vi "Backpressure test.vi"() -> ()   [LabVIEW 2021]
uses:
  typedef/Publisher Configuration.ctl
  typedef/Subscriber Configuration.ctl
  f27365a0-1864-4553-9f92-95bc83607519.vi
  57a9d767-a0aa-4728-95e7-aa61df6a1e2a.vi
  5d6ebc0a-921d-4227-9a00-435e824b8c93.vi
  d8bc2f99-22bc-43ae-b6fa-f8197ccb679b.vi
  1491cca6-a426-4f56-b87d-caac723d0473.vi
  39ed5927-df74-4a57-8dc9-96b021c80492.vi
  bbeb782f-bf74-416e-b0f9-de587b9af98f.vi
  859c98ed-807b-4b96-b06d-d6fb0e9e6f96.vi
  98931993-9e05-4946-a0e8-0782cf58acce.vi
  4db17f17-fbf3-42bc-8837-34dee5865092.vi
  ecbb9208-e776-414e-87f1-19c139091137.vi
  0167b3dc-6f49-4672-b3aa-d51916ebff2c.vi
  84c46a71-3ad6-417c-9aba-be379b5775e6.vi
  233ed9d6-ced9-42df-a9b8-edee980e2fa8.vi
  ff1f2ce0-8d1f-4625-a632-bddccbd44b74.vi
  06a3f26d-2d18-4b18-9314-4c38afe24da5.vi
  564cef77-d045-47f3-b68c-94ab523690b1.vi
  e3fe31ea-c0bd-4811-9f2d-7e19ce1afda0.vi
  23c5baeb-c843-4c9d-b5a5-34d50c9b2511.vi
  92b06e78-0e1e-4219-ba7d-c2e09868a523.vi
  SubVIs/Get Path.vi
  SubVIs/Convert Error.vi
  f27365a0-1864-4553-9f92-95bc83607519.vi/f164bb55-fadc-406a-97d8-e3295a396b46.vi
  SubVIs/Add Error.vi
  Refnum/Raw Publisher to Refnum.vi
  <vilib>/CIF Foundation/CIF Utilities/File/File/File Not Found Error Update.vi
  57a9d767-a0aa-4728-95e7-aa61df6a1e2a.vi/15451e88-64ef-462d-9cc0-58968935b893.vi
  Refnum/Raw Subscriber to Refnum.vi
  Refnum/Raw Publisher from Refnum.vi
  Refnum/Raw Subscriber from Refnum.vi
  1491cca6-a426-4f56-b87d-caac723d0473.vi/f164bb55-fadc-406a-97d8-e3295a396b46.vi
  39ed5927-df74-4a57-8dc9-96b021c80492.vi/15451e88-64ef-462d-9cc0-58968935b893.vi
  98931993-9e05-4946-a0e8-0782cf58acce.vi/f164bb55-fadc-406a-97d8-e3295a396b46.vi
  4db17f17-fbf3-42bc-8837-34dee5865092.vi/15451e88-64ef-462d-9cc0-58968935b893.vi
  84c46a71-3ad6-417c-9aba-be379b5775e6.vi/f164bb55-fadc-406a-97d8-e3295a396b46.vi
  ff1f2ce0-8d1f-4625-a632-bddccbd44b74.vi/15451e88-64ef-462d-9cc0-58968935b893.vi
  564cef77-d045-47f3-b68c-94ab523690b1.vi/f164bb55-fadc-406a-97d8-e3295a396b46.vi
  e3fe31ea-c0bd-4811-9f2d-7e19ce1afda0.vi/15451e88-64ef-462d-9cc0-58968935b893.vi
  <vilib>/Utility/error.llb/Trim Whitespace.vi
  SubVIs/Add Error Core.vi
  <vilib>/CIF Foundation/CIF Utilities/DataTypes/Utilities/Get Element Info of Variant.vi
  SubVIs/Get Type String.vi
  <vilib>/CIF Foundation/CIF Utilities/DataTypes/Utilities/Get JSON Descriptor of Variant.vi
  SubVIs/Convert Error Core.vi
  <vilib>/CIF Foundation/CIF Utilities/File/SubVIs/File Not Found Error Core.vi
  Iceoryx.lvlib
panel:
  out "status":string
  out "pass":bool
  out "error out":errorcluster
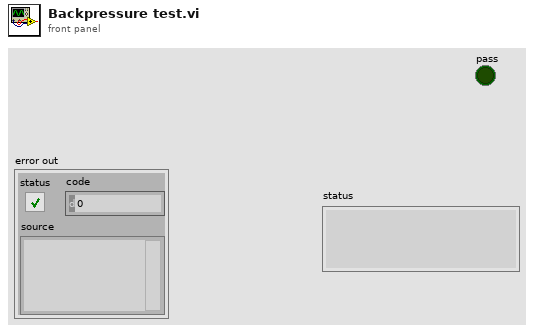
[diagram p1: front panel]
types:
  T1 = typedef "Iceoryx.lvlib/Subscriber Configuration.ctl" = cluster{"Name":string, "Topic":string, "Type":string, "Backpressure":bool}
  T2 = typedef "Iceoryx.lvlib/Publisher Configuration.ctl" = cluster{"Name":string, "Topic":string, "Type":string, "Best Effort Subscribers":u32, "Backpressure Subscribers":u32, "Best Effort Queue Depth":u32, "Backpressure Queue Depth":u32}
  T3 = typedef "Iceoryx.lvlib/Raw Publisher Refnum.ctl" = cluster{"refnum":u64, "Raw Pub":enum8{"rawpub"}}
  T4 = typedef "Iceoryx.lvlib/Raw Subscriber Refnum.ctl" = cluster{"refnum":u64, "Raw Sub":enum8{"rawsub"}}
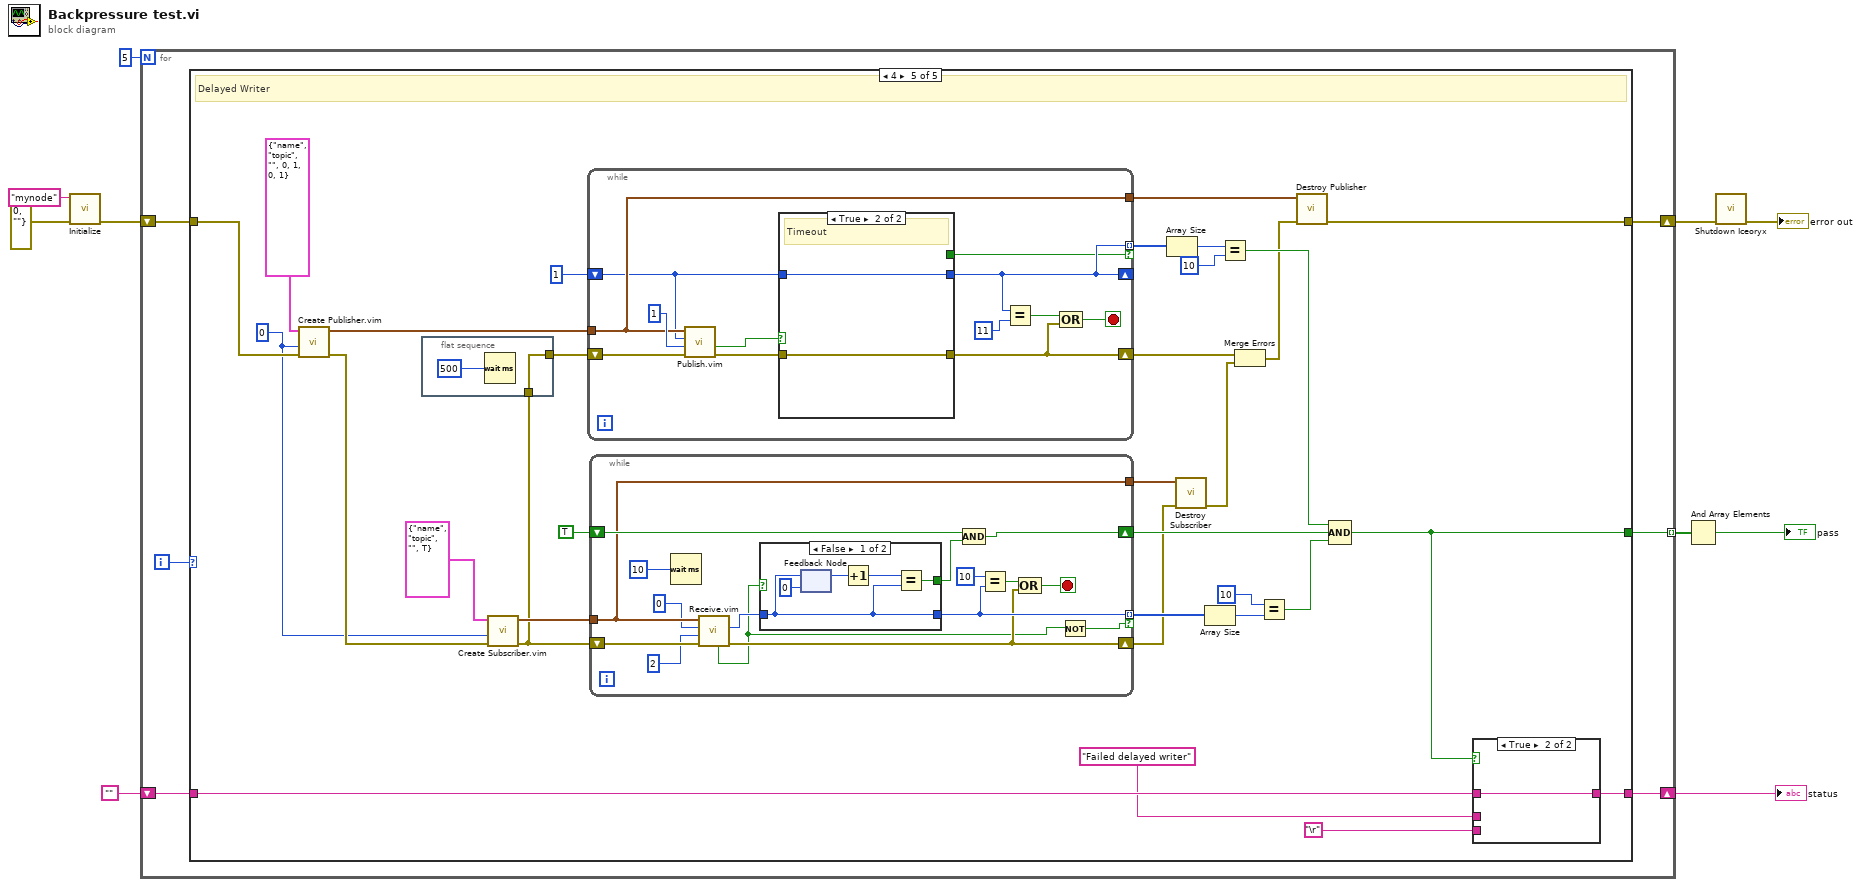
[diagram p0: block diagram]
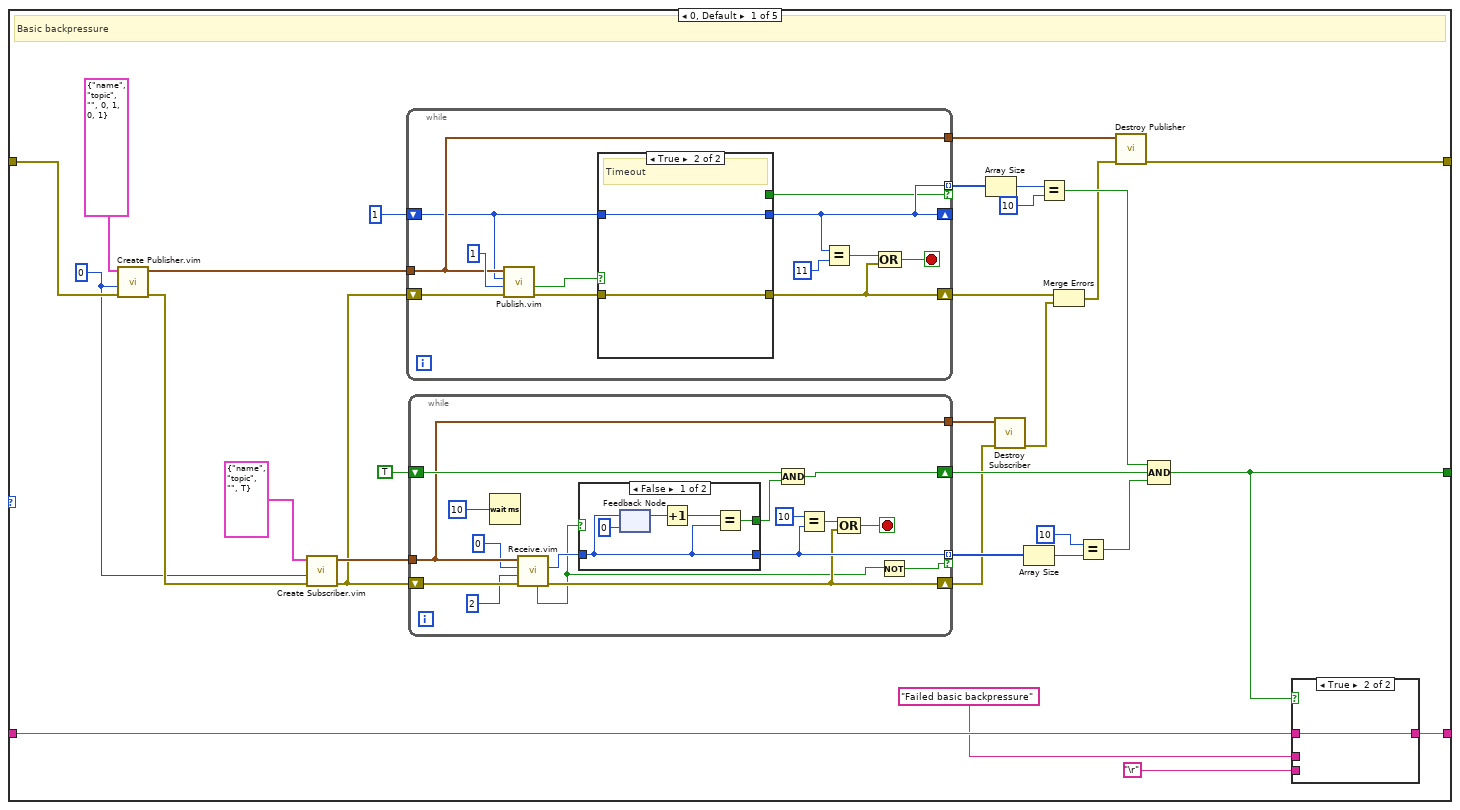
[diagram p2: hidden frame]
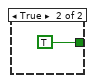
[diagram p3: hidden frame]
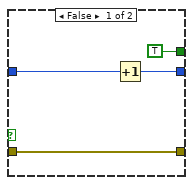
[diagram p4: hidden frame]
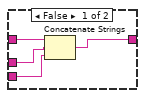
[diagram p5: hidden frame]
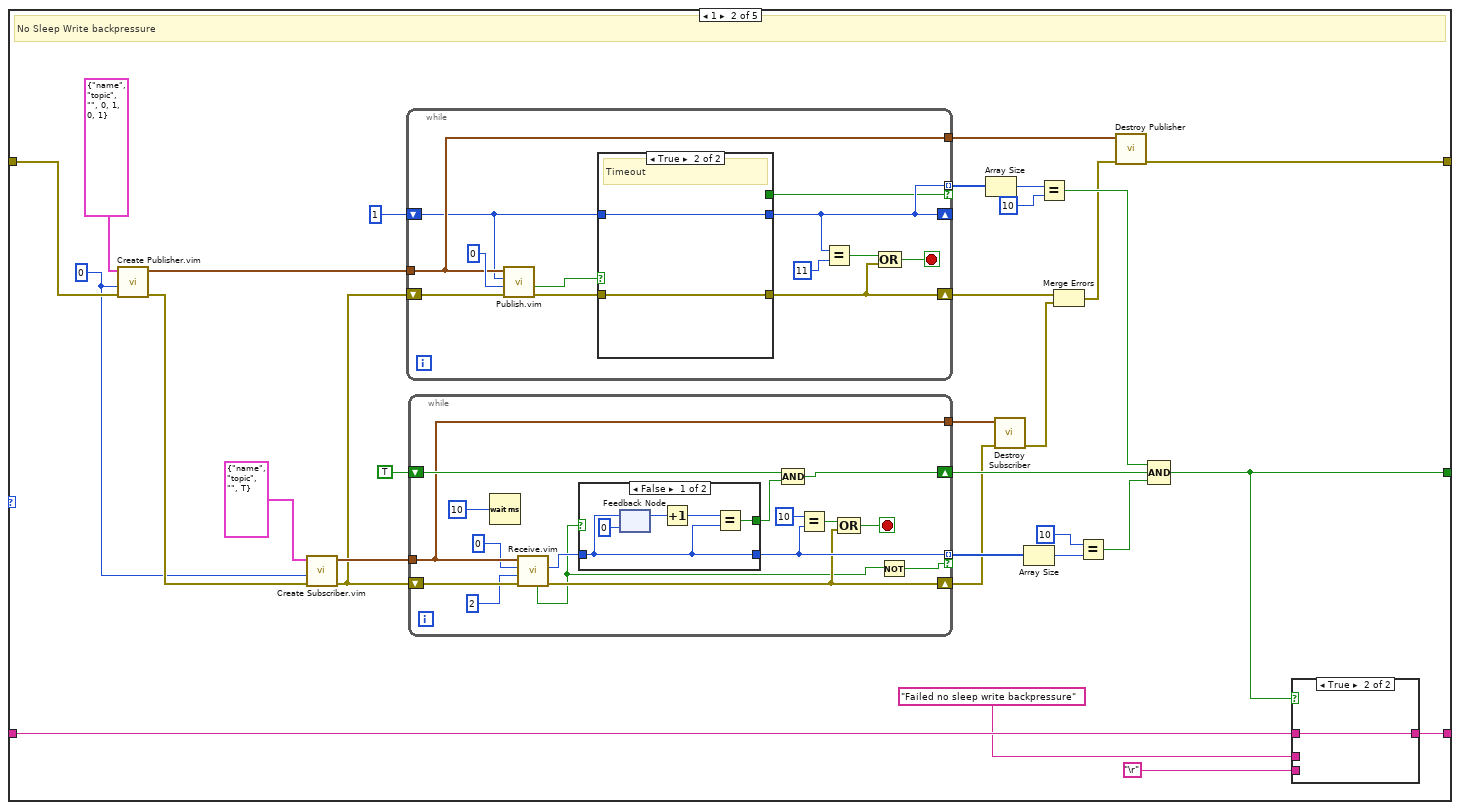
[diagram p6: hidden frame]
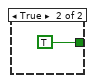
[diagram p7: hidden frame]
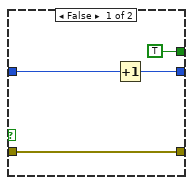
[diagram p8: hidden frame]
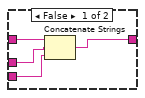
[diagram p9: hidden frame]
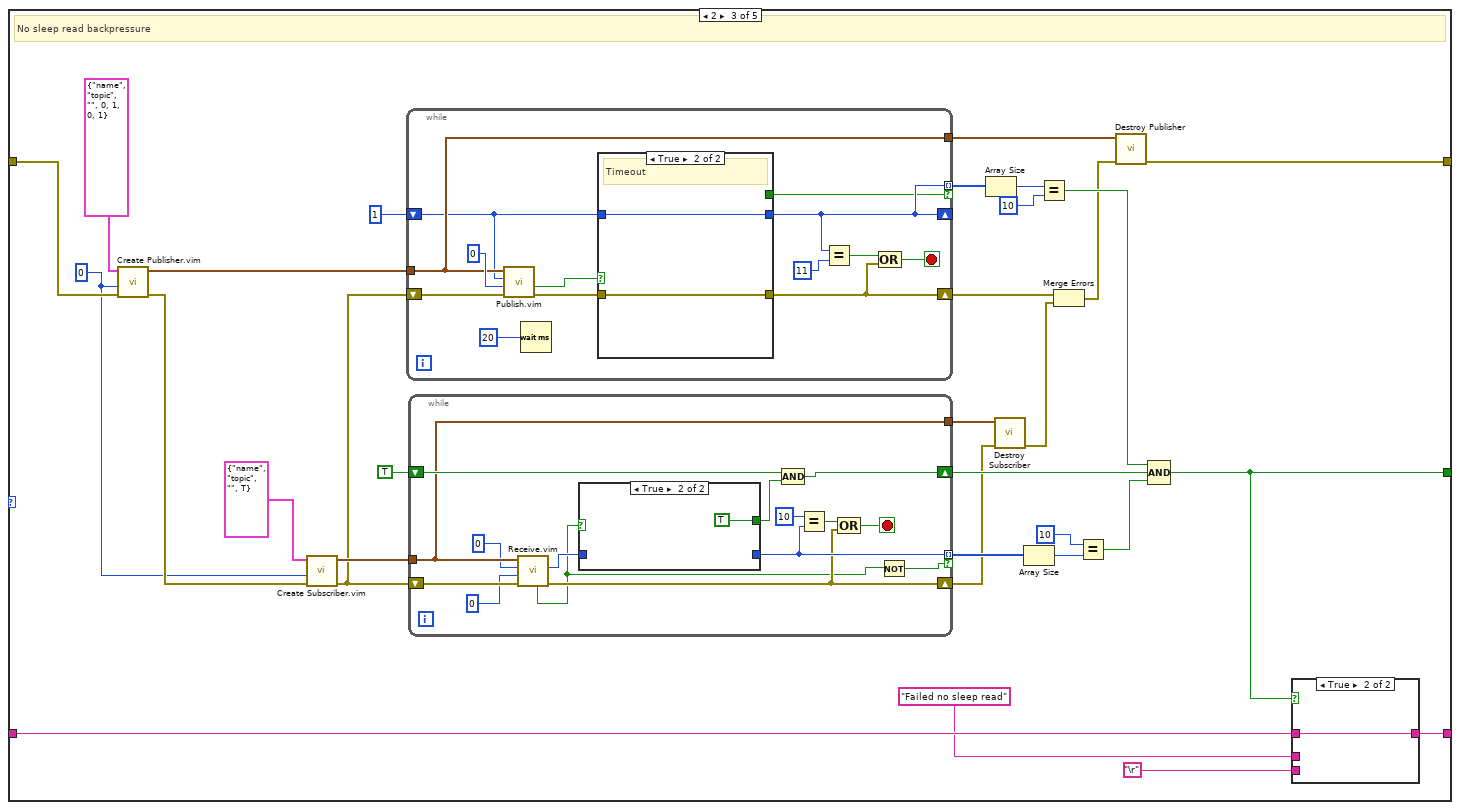
[diagram p10: hidden frame]
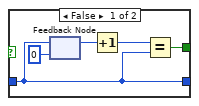
[diagram p11: hidden frame]
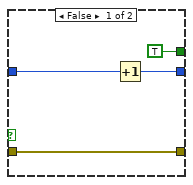
[diagram p12: hidden frame]
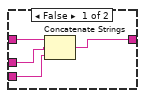
[diagram p13: hidden frame]
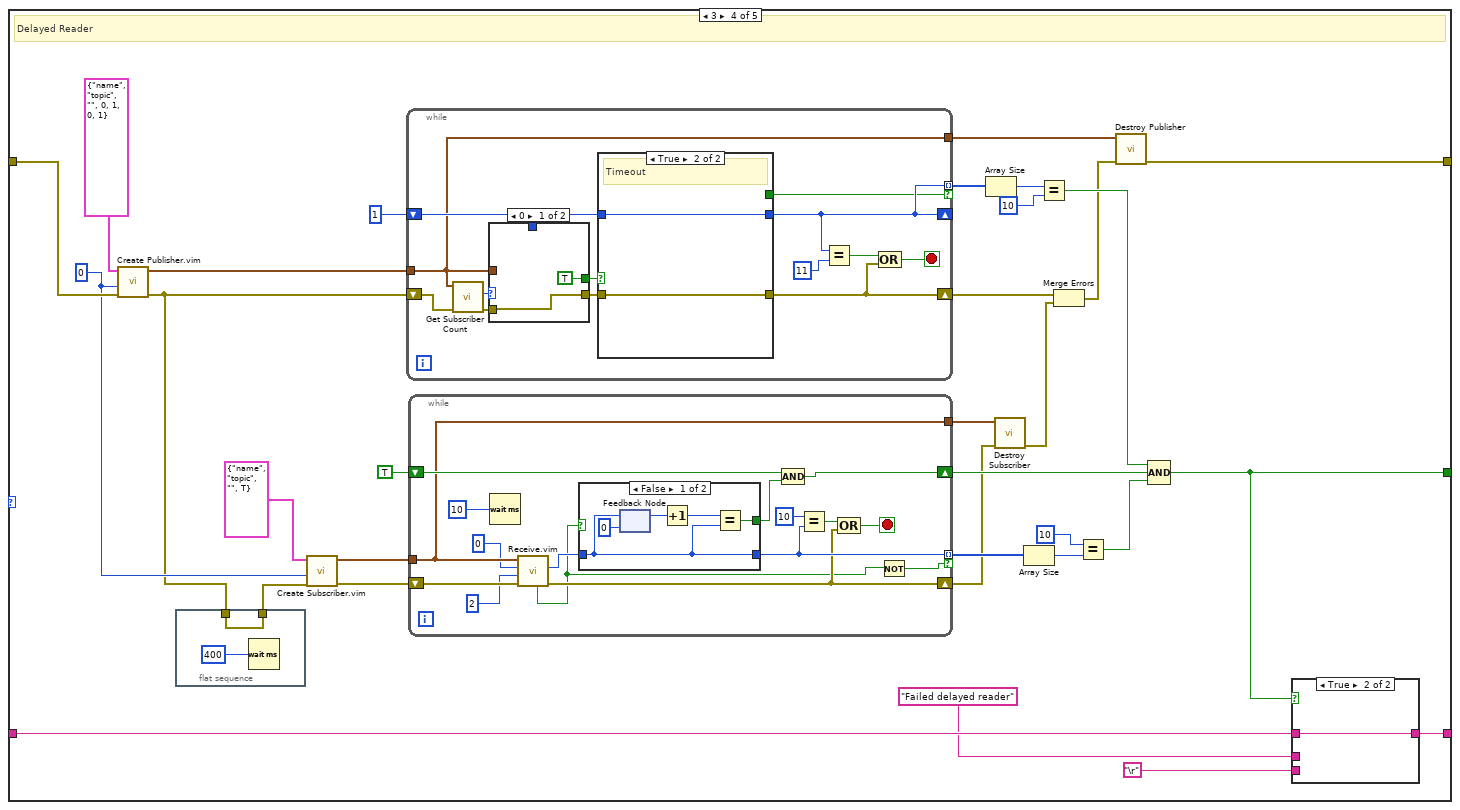
[diagram p14: hidden frame]
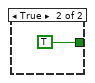
[diagram p15: hidden frame]
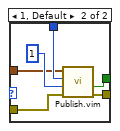
[diagram p16: hidden frame]
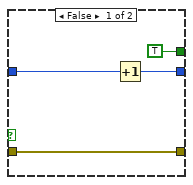
[diagram p17: hidden frame]
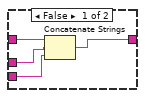
[diagram p18: hidden frame]
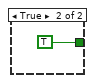
[diagram p19: hidden frame]
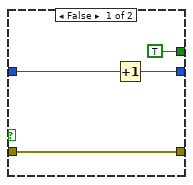
[diagram p20: hidden frame]
diagram:
  n1 = call "Initialize.vi"("error in (no error)"=errorcluster {"status"=FALSE, "code"=0, "source"=""} ("error out"), "Node name"="mynode") -> ("error out"=w4:errorcluster)  [unwired: 9 in]
  n2 = for {
    N: 5 -> [_]
    tunnel: [w16] -> w10 mode=indexing
    shift-right: [w13] -> w6
    shift-left: "" -> [w14]
    shift-right: [w12] -> w2
    shift-left: w4 -> [w11]
    i -> [w15]
    n3 = case shown="4" w15 {
      tunnel: [w35 w111 w187 w264 w352] -> w16
      tunnel: w14 -> [w47 w123 w199 w276 w364]
      tunnel: [w46 w122 w198 w275 w363] -> w13
      tunnel: [w18 w94 w170 w248 w335] -> w12
      tunnel: w11 -> [w30 w106 w182 w259 w347]
      frame 0, Default {
        w24 = 0
        # "Basic backpressure"
        n4 = call "Create Publisher.vim"("error in (no error)"=w30, "Data"=w24, "Publisher Configuration"=T2 {"Name"="name", "Topic"="topic", "Type"="", "Best Effort Subscribers"=0, "Backpressure Subscribers"=1, "Best Effort Queue Depth"=0, "Backpressure Queue Depth"=1}) -> ("error out"=w27:errorcluster, "Publisher Reference"=w28:T3)  [unwired: 6 in, 1 out]
        n5 = call "Create Subscriber.vim"("error in (no error)"=w27, "Data Type"=w24, "Subscriber Configuration"=T1 {"Name"="name", "Topic"="topic", "Type"="", "Backpressure"=TRUE}) -> ("error out"=w17:errorcluster, "Subscriber Reference"=w26:T4)  [unwired: 6 in, 1 out]
        n6 = while {
          tunnel: w28 -> [w72]
          shift-right: [w79] -> w43
          shift-left: w17 -> [w75]
          shift-right: [w77] -> _
          shift-left: 1 ("Data out") -> [w71]
          tunnel: [w77] -> w34 mode=indexing if=w76
          tunnel: [w72] -> w20
          stop <- w78 stop-if-true
          n7 = call "Publish.vim"("error in (no error)"=w75, "Timoeut ms"=i64 1 ("Timeout (ns)"), "Data In"=w71, "Publisher Reference"=w72) -> ("error out"=w70:errorcluster, "Timeout"=w73:bool)  [unwired: 5 in, 1 out]
          n8 = case shown="True" w73 {
            tunnel: w70 -> [w82 w87]
            tunnel: [w82 w87] -> w79
            tunnel: w71 -> [w85 w86]
            tunnel: [w84 w86] -> w77
            tunnel: [TRUE _] -> w76
            frame False {
              n9 = Increment(x=w85) -> (x+1=w84:i32)
            }
            frame True {
              # "Timeout"
            }
          }
          n10 = Equal?(x=w77, y=11) -> (x = y?=w80:bool)
          n11 = Compound Arithmetic op=OR(w80, w79) -> (w78:bool)
        }
        n12 = while {
          shift-right: [w60] -> w37
          shift-left: TRUE -> [w62]
          shift-right: [w53] -> w22
          shift-left: w17 -> [w55]
          tunnel: [w59] -> w40 mode=indexing if=w49
          tunnel: w26 -> [w54]
          tunnel: [w54] -> w23
          stop <- w56 stop-if-true
          n13 = Wait (ms)(milliseconds to wait=u32 10) -> ()  [unwired: 1 out]
          n14 = call "Receive.vim"("error in (no error)"=w55, "Timoeut ms"=2, "Data In"=0, "Subscriber Reference"=w54) -> ("error out"=w53:errorcluster, "Data Out"=w50:i32, "Timeout"=w48:bool)  [unwired: 4 in, 1 out]
          n15 = case shown="False" w48 {
            tunnel: w50 -> [w64 _]
            tunnel: [w65 TRUE] -> w61
            tunnel: [w64 _] -> w59
            frame False {
              n16 = feedback #1(0 ("Data out")) -> (w67:i32)
              n17 = feedback-in #1(w64) -> ()
              n18 = Increment(x=w67) -> (x+1=w66:i32)
              n19 = Equal?(x=w66, y=w64) -> (x = y?=w65:bool)
            }
            frame True {
            }
          }
          n20 = Compound Arithmetic op=AND(w62, w61) -> (w60:bool)
          n21 = Equal?(x=10, y=w59) -> (x = y?=w57:bool)
          n22 = Compound Arithmetic op=OR(w57, w53) -> (w56:bool)
          n23 = Not(x=w48) -> (.not. x?=w49:bool)
        }
        n24 = Array Size(array=w34) -> (size(s)=w33:i32)
        n25 = call "Destroy Subscriber.vi"("error in (no error)"=w22, "Subscriber Reference"=w23) -> ("error out"=w21:errorcluster)  [unwired: 9 in]
        n26 = Array Size(array=w40) -> (size(s)=w39:i32)
        n27 = Equal?(x=w33, y=10 ("x")) -> (x = y?=w31:bool)
        n28 = Merge Errors(w43, w21) -> (w19:errorcluster)
        n29 = Equal?(x=10, y=w39) -> (x = y?=w36:bool)
        n30 = call "Destroy Publisher.vi"("error in (no error)"=w19, "Publisher Reference"=w20) -> ("error out"=w18:errorcluster)  [unwired: 9 in]
        n31 = Compound Arithmetic op=AND(w31, w37, w36) -> (w35:bool)
        n32 = case shown="True" w35 {
          tunnel: w47 -> [w91 w92]
          tunnel: [w88 w92] -> w46
          tunnel: "Failed basic backpressure" -> [w90 _]
          tunnel: "\r" -> [w89 _]
          frame False {
            n33 = Concatenate Strings(w91, w90, w89) -> (w88:string)
          }
          frame True {
          }
        }
      }
      frame 1 {
        w100 = 0
        # "No Sleep Write backpressure"
        n34 = call "Create Publisher.vim"("error in (no error)"=w106, "Data"=w100, "Publisher Configuration"=T2 {"Name"="name", "Topic"="topic", "Type"="", "Best Effort Subscribers"=0, "Backpressure Subscribers"=1, "Best Effort Queue Depth"=0, "Backpressure Queue Depth"=1}) -> ("error out"=w103:errorcluster, "Publisher Reference"=w104:T3)  [unwired: 6 in, 1 out]
        n35 = call "Create Subscriber.vim"("error in (no error)"=w103, "Data Type"=w100, "Subscriber Configuration"=T1 {"Name"="name", "Topic"="topic", "Type"="", "Backpressure"=TRUE}) -> ("error out"=w93:errorcluster, "Subscriber Reference"=w102:T4)  [unwired: 6 in, 1 out]
        n36 = while {
          tunnel: w104 -> [w148]
          shift-right: [w155] -> w119
          shift-left: w93 -> [w151]
          shift-right: [w153] -> _
          shift-left: 1 ("Data out") -> [w147]
          tunnel: [w153] -> w110 mode=indexing if=w152
          tunnel: [w148] -> w96
          stop <- w154 stop-if-true
          n37 = call "Publish.vim"("error in (no error)"=w151, "Timoeut ms"=i64 0 ("Timeout (ns)"), "Data In"=w147, "Publisher Reference"=w148) -> ("error out"=w146:errorcluster, "Timeout"=w149:bool)  [unwired: 5 in, 1 out]
          n38 = case shown="True" w149 {
            tunnel: w146 -> [w158 w163]
            tunnel: [w158 w163] -> w155
            tunnel: w147 -> [w161 w162]
            tunnel: [w160 w162] -> w153
            tunnel: [TRUE _] -> w152
            frame False {
              n39 = Increment(x=w161) -> (x+1=w160:i32)
            }
            frame True {
              # "Timeout"
            }
          }
          n40 = Equal?(x=w153, y=11) -> (x = y?=w156:bool)
          n41 = Compound Arithmetic op=OR(w156, w155) -> (w154:bool)
        }
        n42 = while {
          shift-right: [w136] -> w113
          shift-left: TRUE -> [w138]
          shift-right: [w129] -> w98
          shift-left: w93 -> [w131]
          tunnel: [w135] -> w116 mode=indexing if=w125
          tunnel: w102 -> [w130]
          tunnel: [w130] -> w99
          stop <- w132 stop-if-true
          n43 = Wait (ms)(milliseconds to wait=u32 10) -> ()  [unwired: 1 out]
          n44 = call "Receive.vim"("error in (no error)"=w131, "Timoeut ms"=2, "Data In"=0, "Subscriber Reference"=w130) -> ("error out"=w129:errorcluster, "Data Out"=w126:i32, "Timeout"=w124:bool)  [unwired: 4 in, 1 out]
          n45 = case shown="False" w124 {
            tunnel: w126 -> [w140 _]
            tunnel: [w141 TRUE] -> w137
            tunnel: [w140 _] -> w135
            frame False {
              n46 = feedback #2(0 ("Data out")) -> (w143:i32)
              n47 = feedback-in #2(w140) -> ()
              n48 = Increment(x=w143) -> (x+1=w142:i32)
              n49 = Equal?(x=w142, y=w140) -> (x = y?=w141:bool)
            }
            frame True {
            }
          }
          n50 = Compound Arithmetic op=AND(w138, w137) -> (w136:bool)
          n51 = Equal?(x=10, y=w135) -> (x = y?=w133:bool)
          n52 = Compound Arithmetic op=OR(w133, w129) -> (w132:bool)
          n53 = Not(x=w124) -> (.not. x?=w125:bool)
        }
        n54 = Array Size(array=w110) -> (size(s)=w109:i32)
        n55 = call "Destroy Subscriber.vi"("error in (no error)"=w98, "Subscriber Reference"=w99) -> ("error out"=w97:errorcluster)  [unwired: 9 in]
        n56 = Array Size(array=w116) -> (size(s)=w115:i32)
        n57 = Equal?(x=w109, y=10 ("x")) -> (x = y?=w107:bool)
        n58 = Merge Errors(w119, w97) -> (w95:errorcluster)
        n59 = Equal?(x=10, y=w115) -> (x = y?=w112:bool)
        n60 = call "Destroy Publisher.vi"("error in (no error)"=w95, "Publisher Reference"=w96) -> ("error out"=w94:errorcluster)  [unwired: 9 in]
        n61 = Compound Arithmetic op=AND(w107, w113, w112) -> (w111:bool)
        n62 = case shown="True" w111 {
          tunnel: w123 -> [w167 w168]
          tunnel: [w164 w168] -> w122
          tunnel: "Failed no sleep write backpressure" -> [w166 _]
          tunnel: "\r" -> [w165 _]
          frame False {
            n63 = Concatenate Strings(w167, w166, w165) -> (w164:string)
          }
          frame True {
          }
        }
      }
      frame 2 {
        w176 = 0
        # "No sleep read backpressure"
        n64 = call "Create Publisher.vim"("error in (no error)"=w182, "Data"=w176, "Publisher Configuration"=T2 {"Name"="name", "Topic"="topic", "Type"="", "Best Effort Subscribers"=0, "Backpressure Subscribers"=1, "Best Effort Queue Depth"=0, "Backpressure Queue Depth"=1}) -> ("error out"=w179:errorcluster, "Publisher Reference"=w180:T3)  [unwired: 6 in, 1 out]
        n65 = call "Create Subscriber.vim"("error in (no error)"=w179, "Data Type"=w176, "Subscriber Configuration"=T1 {"Name"="name", "Topic"="topic", "Type"="", "Backpressure"=TRUE}) -> ("error out"=w169:errorcluster, "Subscriber Reference"=w178:T4)  [unwired: 6 in, 1 out]
        n66 = while {
          tunnel: w180 -> [w224]
          shift-right: [w231] -> w195
          shift-left: w169 -> [w227]
          shift-right: [w229] -> _
          shift-left: 1 ("Data out") -> [w223]
          tunnel: [w229] -> w186 mode=indexing if=w228
          tunnel: [w224] -> w172
          stop <- w230 stop-if-true
          n67 = call "Publish.vim"("error in (no error)"=w227, "Timoeut ms"=i64 0 ("Timeout (ns)"), "Data In"=w223, "Publisher Reference"=w224) -> ("error out"=w222:errorcluster, "Timeout"=w225:bool)  [unwired: 5 in, 1 out]
          n68 = Wait (ms)(milliseconds to wait=u32 20) -> ()  [unwired: 1 out]
          n69 = case shown="True" w225 {
            tunnel: w222 -> [w234 w239]
            tunnel: [w234 w239] -> w231
            tunnel: w223 -> [w237 w238]
            tunnel: [w236 w238] -> w229
            tunnel: [TRUE _] -> w228
            frame False {
              n70 = Increment(x=w237) -> (x+1=w236:i32)
            }
            frame True {
              # "Timeout"
            }
          }
          n71 = Equal?(x=w229, y=11) -> (x = y?=w232:bool)
          n72 = Compound Arithmetic op=OR(w232, w231) -> (w230:bool)
        }
        n73 = while {
          shift-right: [w212] -> w189
          shift-left: TRUE -> [w214]
          shift-right: [w205] -> w174
          shift-left: w169 -> [w207]
          tunnel: [w211] -> w192 mode=indexing if=w201
          tunnel: w178 -> [w206]
          tunnel: [w206] -> w175
          stop <- w208 stop-if-true
          n74 = call "Receive.vim"("error in (no error)"=w207, "Timoeut ms"=0, "Data In"=0, "Subscriber Reference"=w206) -> ("error out"=w205:errorcluster, "Data Out"=w202:i32, "Timeout"=w200:bool)  [unwired: 4 in, 1 out]
          n75 = case shown="True" w200 {
            tunnel: w202 -> [w215 _]
            tunnel: [w216 TRUE] -> w213
            tunnel: [w215 _] -> w211
            frame False {
              n76 = feedback #3(0 ("Data out")) -> (w218:i32)
              n77 = feedback-in #3(w215) -> ()
              n78 = Increment(x=w218) -> (x+1=w217:i32)
              n79 = Equal?(x=w217, y=w215) -> (x = y?=w216:bool)
            }
            frame True {
            }
          }
          n80 = Compound Arithmetic op=AND(w214, w213) -> (w212:bool)
          n81 = Equal?(x=10, y=w211) -> (x = y?=w209:bool)
          n82 = Compound Arithmetic op=OR(w209, w205) -> (w208:bool)
          n83 = Not(x=w200) -> (.not. x?=w201:bool)
        }
        n84 = Array Size(array=w186) -> (size(s)=w185:i32)
        n85 = call "Destroy Subscriber.vi"("error in (no error)"=w174, "Subscriber Reference"=w175) -> ("error out"=w173:errorcluster)  [unwired: 9 in]
        n86 = Array Size(array=w192) -> (size(s)=w191:i32)
        n87 = Equal?(x=w185, y=10 ("x")) -> (x = y?=w183:bool)
        n88 = Merge Errors(w195, w173) -> (w171:errorcluster)
        n89 = Equal?(x=10, y=w191) -> (x = y?=w188:bool)
        n90 = call "Destroy Publisher.vi"("error in (no error)"=w171, "Publisher Reference"=w172) -> ("error out"=w170:errorcluster)  [unwired: 9 in]
        n91 = Compound Arithmetic op=AND(w183, w189, w188) -> (w187:bool)
        n92 = case shown="True" w187 {
          tunnel: w199 -> [w243 w244]
          tunnel: [w240 w244] -> w198
          tunnel: "Failed no sleep read" -> [w242 _]
          tunnel: "\r" -> [w241 _]
          frame False {
            n93 = Concatenate Strings(w243, w242, w241) -> (w240:string)
          }
          frame True {
          }
        }
      }
      frame 3 {
        w254 = 0
        # "Delayed Reader"
        n94 = call "Create Publisher.vim"("error in (no error)"=w259, "Data"=w254, "Publisher Configuration"=T2 {"Name"="name", "Topic"="topic", "Type"="", "Best Effort Subscribers"=0, "Backpressure Subscribers"=1, "Best Effort Queue Depth"=0, "Backpressure Queue Depth"=1}) -> ("error out"=w245:errorcluster, "Publisher Reference"=w257:T3)  [unwired: 6 in, 1 out]
        n95 = flat-sequence {
          tunnel: w245 -> [w278]
          tunnel: [w278] -> w246
          frame #0 {
            n96 = Wait (ms)(milliseconds to wait=u32 400) -> ()  [unwired: 1 out]
          }
        }
        n97 = call "Create Subscriber.vim"("error in (no error)"=w246, "Data Type"=w254, "Subscriber Configuration"=T1 {"Name"="name", "Topic"="topic", "Type"="", "Backpressure"=TRUE}) -> ("error out"=w247:errorcluster, "Subscriber Reference"=w256:T4)  [unwired: 6 in, 1 out]
        n98 = while {
          tunnel: w257 -> [w304]
          shift-right: [w311] -> w272
          shift-left: w245 -> [w303]
          shift-right: [w309] -> _
          shift-left: 1 ("Data out") -> [w306]
          tunnel: [w309] -> w263 mode=indexing if=w308
          tunnel: [w304] -> w250
          stop <- w310 stop-if-true
          n99 = call "Get Subscriber Count.vi"("error in (no error)"=w303, "Publisher Reference"=w304) -> ("error out"=w302:errorcluster, "Backpressure"=w301:u32)  [unwired: 7 in, 1 out]
          n100 = case shown="0" w301 {
            tunnel: [TRUE ("Timeout") w320] -> w307
            tunnel: w306 -> [_ w319]
            tunnel: [w315 w318] -> w305
            tunnel: w304 -> [_ w317]
            tunnel: w302 -> [w315 w316]
            frame 0 {
            }
            frame 1, Default {
              n101 = call "Publish.vim"("error in (no error)"=w316, "Timoeut ms"=i64 1 ("Timeout (ns)"), "Data In"=w319, "Publisher Reference"=w317) -> ("error out"=w318:errorcluster, "Timeout"=w320:bool)  [unwired: 5 in, 1 out]
            }
          }
          n102 = case shown="True" w307 {
            tunnel: w305 -> [w322 w327]
            tunnel: [w322 w327] -> w311
            tunnel: w306 -> [w325 w326]
            tunnel: [w324 w326] -> w309
            tunnel: [TRUE _] -> w308
            frame False {
              n103 = Increment(x=w325) -> (x+1=w324:i32)
            }
            frame True {
              # "Timeout"
            }
          }
          n104 = Equal?(x=w309, y=11) -> (x = y?=w312:bool)
          n105 = Compound Arithmetic op=OR(w312, w311) -> (w310:bool)
        }
        n106 = while {
          shift-right: [w291] -> w266
          shift-left: TRUE -> [w293]
          shift-right: [w284] -> w252
          shift-left: w247 -> [w286]
          tunnel: [w290] -> w269 mode=indexing if=w280
          tunnel: w256 -> [w285]
          tunnel: [w285] -> w253
          stop <- w287 stop-if-true
          n107 = Wait (ms)(milliseconds to wait=u32 10) -> ()  [unwired: 1 out]
          n108 = call "Receive.vim"("error in (no error)"=w286, "Timoeut ms"=2, "Data In"=0, "Subscriber Reference"=w285) -> ("error out"=w284:errorcluster, "Data Out"=w281:i32, "Timeout"=w279:bool)  [unwired: 4 in, 1 out]
          n109 = case shown="False" w279 {
            tunnel: w281 -> [w295 _]
            tunnel: [w296 TRUE] -> w292
            tunnel: [w295 _] -> w290
            frame False {
              n110 = feedback #4(0 ("Data out")) -> (w298:i32)
              n111 = feedback-in #4(w295) -> ()
              n112 = Increment(x=w298) -> (x+1=w297:i32)
              n113 = Equal?(x=w297, y=w295) -> (x = y?=w296:bool)
            }
            frame True {
            }
          }
          n114 = Compound Arithmetic op=AND(w293, w292) -> (w291:bool)
          n115 = Equal?(x=10, y=w290) -> (x = y?=w288:bool)
          n116 = Compound Arithmetic op=OR(w288, w284) -> (w287:bool)
          n117 = Not(x=w279) -> (.not. x?=w280:bool)
        }
        n118 = Array Size(array=w263) -> (size(s)=w262:i32)
        n119 = call "Destroy Subscriber.vi"("error in (no error)"=w252, "Subscriber Reference"=w253) -> ("error out"=w251:errorcluster)  [unwired: 9 in]
        n120 = Array Size(array=w269) -> (size(s)=w268:i32)
        n121 = Equal?(x=w262, y=10 ("x")) -> (x = y?=w260:bool)
        n122 = Merge Errors(w272, w251) -> (w249:errorcluster)
        n123 = Equal?(x=10, y=w268) -> (x = y?=w265:bool)
        n124 = call "Destroy Publisher.vi"("error in (no error)"=w249, "Publisher Reference"=w250) -> ("error out"=w248:errorcluster)  [unwired: 9 in]
        n125 = Compound Arithmetic op=AND(w260, w266, w265) -> (w264:bool)
        n126 = case shown="True" w264 {
          tunnel: w276 -> [w331 w332]
          tunnel: [w328 w332] -> w275
          tunnel: "Failed delayed reader" -> [w330 _]
          tunnel: "\r" -> [w329 _]
          frame False {
            n127 = Concatenate Strings(w331, w330, w329) -> (w328:string)
          }
          frame True {
          }
        }
      }
      frame 4 {
        w341 = 0
        # "Delayed Writer"
        n128 = call "Create Publisher.vim"("error in (no error)"=w347, "Data"=w341, "Publisher Configuration"=T2 {"Name"="name", "Topic"="topic", "Type"="", "Best Effort Subscribers"=0, "Backpressure Subscribers"=1, "Best Effort Queue Depth"=0, "Backpressure Queue Depth"=1}) -> ("error out"=w344:errorcluster, "Publisher Reference"=w345:T3)  [unwired: 6 in, 1 out]
        n129 = flat-sequence {
          tunnel: [w365] -> w333
          tunnel: w334 -> [w365]
          frame #0 {
            n130 = Wait (ms)(milliseconds to wait=u32 500) -> ()  [unwired: 1 out]
          }
        }
        n131 = call "Create Subscriber.vim"("error in (no error)"=w344, "Data Type"=w341, "Subscriber Configuration"=T1 {"Name"="name", "Topic"="topic", "Type"="", "Backpressure"=TRUE}) -> ("error out"=w334:errorcluster, "Subscriber Reference"=w343:T4)  [unwired: 6 in, 1 out]
        n132 = while {
          tunnel: w345 -> [w391]
          shift-right: [w398] -> w360
          shift-left: w333 -> [w394]
          shift-right: [w396] -> _
          shift-left: 1 ("Data out") -> [w390]
          tunnel: [w396] -> w351 mode=indexing if=w395
          tunnel: [w391] -> w337
          stop <- w397 stop-if-true
          n133 = call "Publish.vim"("error in (no error)"=w394, "Timoeut ms"=i64 1 ("Timeout (ns)"), "Data In"=w390, "Publisher Reference"=w391) -> ("error out"=w389:errorcluster, "Timeout"=w392:bool)  [unwired: 5 in, 1 out]
          n134 = case shown="True" w392 {
            tunnel: w389 -> [w401 w406]
            tunnel: [w401 w406] -> w398
            tunnel: w390 -> [w404 w405]
            tunnel: [w403 w405] -> w396
            tunnel: [TRUE _] -> w395
            frame False {
              n135 = Increment(x=w404) -> (x+1=w403:i32)
            }
            frame True {
              # "Timeout"
            }
          }
          n136 = Equal?(x=w396, y=11) -> (x = y?=w399:bool)
          n137 = Compound Arithmetic op=OR(w399, w398) -> (w397:bool)
        }
        n138 = while {
          shift-right: [w379] -> w354
          shift-left: TRUE -> [w381]
          shift-right: [w372] -> w339
          shift-left: w334 -> [w374]
          tunnel: [w378] -> w357 mode=indexing if=w368
          tunnel: w343 -> [w373]
          tunnel: [w373] -> w340
          stop <- w375 stop-if-true
          n139 = Wait (ms)(milliseconds to wait=u32 10) -> ()  [unwired: 1 out]
          n140 = call "Receive.vim"("error in (no error)"=w374, "Timoeut ms"=2, "Data In"=0, "Subscriber Reference"=w373) -> ("error out"=w372:errorcluster, "Data Out"=w369:i32, "Timeout"=w367:bool)  [unwired: 4 in, 1 out]
          n141 = case shown="False" w367 {
            tunnel: w369 -> [w383 _]
            tunnel: [w384 TRUE] -> w380
            tunnel: [w383 _] -> w378
            frame False {
              n142 = feedback #5(0 ("Data out")) -> (w386:i32)
              n143 = feedback-in #5(w383) -> ()
              n144 = Increment(x=w386) -> (x+1=w385:i32)
              n145 = Equal?(x=w385, y=w383) -> (x = y?=w384:bool)
            }
            frame True {
            }
          }
          n146 = Compound Arithmetic op=AND(w381, w380) -> (w379:bool)
          n147 = Equal?(x=10, y=w378) -> (x = y?=w376:bool)
          n148 = Compound Arithmetic op=OR(w376, w372) -> (w375:bool)
          n149 = Not(x=w367) -> (.not. x?=w368:bool)
        }
        n150 = Array Size(array=w351) -> (size(s)=w350:i32)
        n151 = call "Destroy Subscriber.vi"("error in (no error)"=w339, "Subscriber Reference"=w340) -> ("error out"=w338:errorcluster)  [unwired: 9 in]
        n152 = Array Size(array=w357) -> (size(s)=w356:i32)
        n153 = Equal?(x=w350, y=10 ("x")) -> (x = y?=w348:bool)
        n154 = Merge Errors(w360, w338) -> (w336:errorcluster)
        n155 = Equal?(x=10, y=w356) -> (x = y?=w353:bool)
        n156 = call "Destroy Publisher.vi"("error in (no error)"=w336, "Publisher Reference"=w337) -> ("error out"=w335:errorcluster)  [unwired: 9 in]
        n157 = Compound Arithmetic op=AND(w348, w354, w353) -> (w352:bool)
        n158 = case shown="True" w352 {
          tunnel: w364 -> [w410 w411]
          tunnel: [w407 w411] -> w363
          tunnel: "Failed delayed writer" -> [w409 _]
          tunnel: "\r" -> [w408 _]
          frame False {
            n159 = Concatenate Strings(w410, w409, w408) -> (w407:string)
          }
          frame True {
          }
        }
      }
    }
  }
  "status" <- w6
  n160 = And Array Elements(Boolean array=w10) -> (logical AND=→"pass":bool)
  n161 = call "Shutdown Iceoryx.vi"("error in (no error)"=w2) -> ("error out"=→"error out":errorcluster)  [unwired: 10 in]
